vi "VM Spy - Dialog - Context Info.vi"(11 "VC Handle":T1=-1) -> (0 "update":bool)   [LabVIEW 2021]
doc: "::: CalcExpress Toolkit :::\nCopyright (c) 2000-2026 Konstantin Shifershteyn. All rights reserved."
uses:
  vi.lib/addons/CalcExpress/cetypes.llb/VarMan Context Life Time.ctl
  vi.lib/addons/CalcExpress/cetypes.llb/VarMan Variable Context Handle.ctl
panel:
  in  "calc size":bool
  in  "size utits":enum16{"Bytes", "KB", "MB"}(ring)
  out "Intended lifetime":T2
  out "used memory":dbl format="%#.3f"
  in  "destroy":bool
  in  "open VI":bool
  out "VI state":string
  out "Creator":string
  in  "close":bool
  in  "rename":bool
  out "Context name":string
  out "Context handle":i32=-1
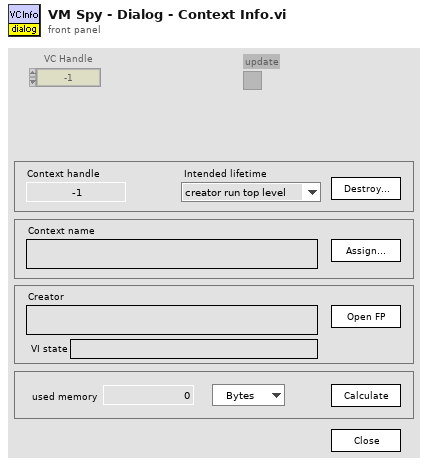
[diagram p1: front panel]
types:
  T1 = typedef "VarMan Variable Context Handle.ctl" = i32
  T2 = typedef "VarMan Context Life Time.ctl" = enum32{"creator run top level", "creator running ", "creator in memory", "untill closed"}
  T3 = enum32{"Bad", "Idle", "Run top level", "Running"}
  T4 = typedef "eventvkey.ctl" = enum16{"ASCII", "Enter", "Return", "Shift", "Ctrl", "Alt", "Cmd", "Opt", "Caps", "NumLock", "Clear", "Break", "Up", "Down", "Left", "Right", "Insert", "Delete", "Home", "End", "PageUp", "PageDown", "Escape", "Help", "Pause", "ScrollLock", "F1", "F2", "F3", "F4", "F5", "F6", "F7", "F8", "F9", "F10", "F11", "F12", "F13", "F14", "F15", "F16", "F17", "F18", "F19", "F20", "F21", "F22", "F23", "F24", "Play", "VolumeUp", "VolumeDown", "Mute", "Two Byte Char"}
  T5 = cluster{"Shift":bool, "Ctrl":bool, "Alt":bool, "Cmd":bool, "Opt":bool}
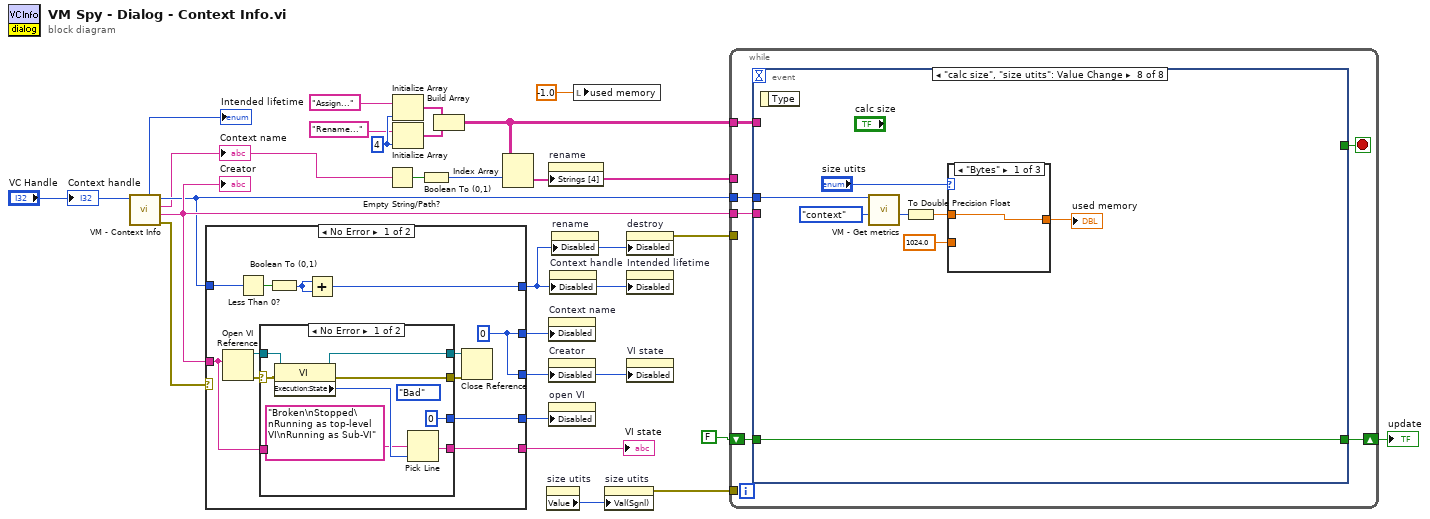
[diagram p0: block diagram]
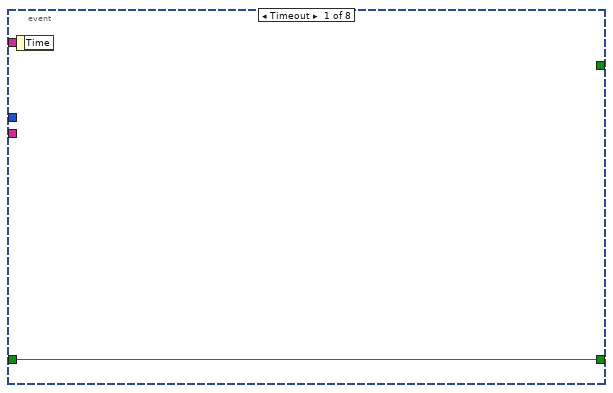
[diagram p2: hidden frame]
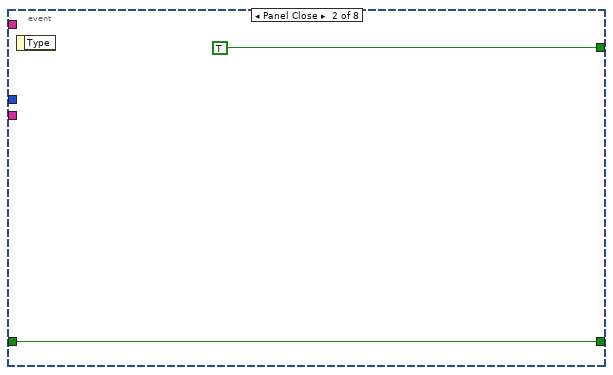
[diagram p3: hidden frame]
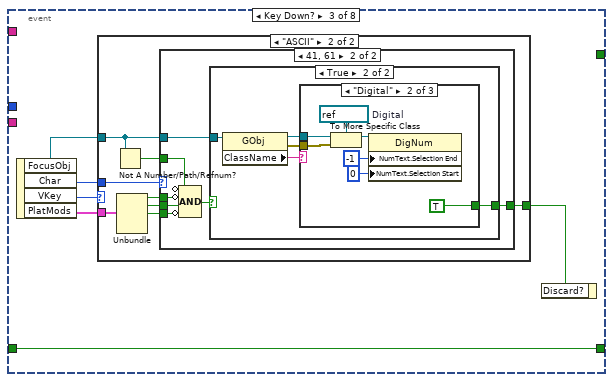
[diagram p4: hidden frame]
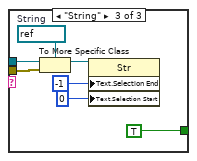
[diagram p9: hidden frame]
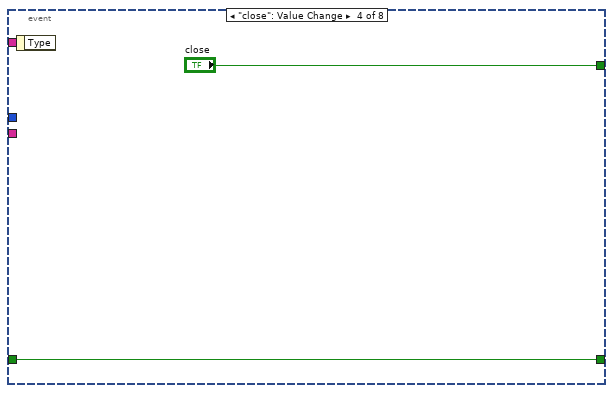
[diagram p10: hidden frame]
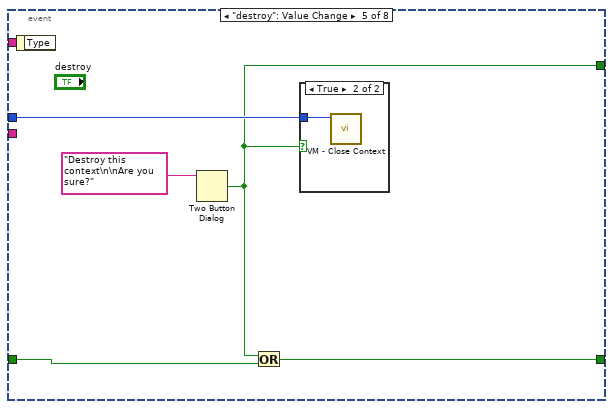
[diagram p11: hidden frame]
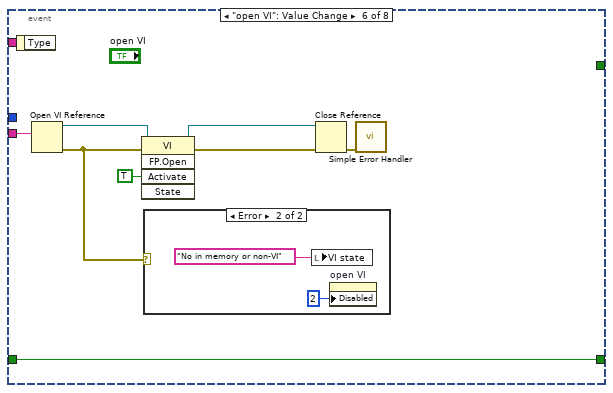
[diagram p13: hidden frame]
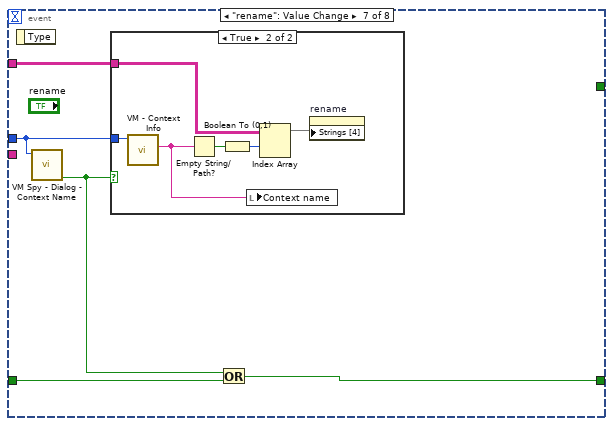
[diagram p15: hidden frame]
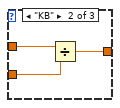
[diagram p17: hidden frame]
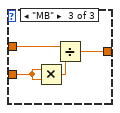
[diagram p18: hidden frame]
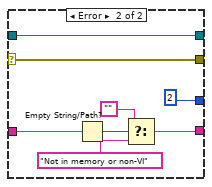
[diagram p19: hidden frame]
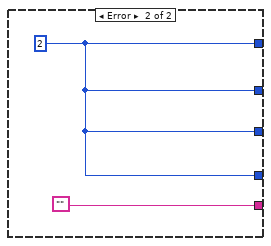
[diagram p20: hidden frame]
diagram:
  w15 = 4 ("dimension size")
  n1 = call "VM - Context Info.vi"("VC Handle"="VC Handle") -> ("error out"=w26:errorcluster, "Creator"=w20:string, "VC Name"=w16:string, "dup VC Handle"=w19:T1, "context life time"=→"Intended lifetime":T2)  [unwired: 6 in]
  "Context name" <- w16
  "Creator" <- w20
  n2 = case shown="No Error" w26 {
    tunnel: w19 -> [w35 _]
    tunnel: w20 -> [w28 _]
    tunnel: [w36 w55] -> w17
    tunnel: [w27 w55] -> w21
    tunnel: [w32 w55] -> w25
    tunnel: [w31 ""] -> w24
    tunnel: [w27 w55] -> w18
    frame No Error {
      w27 = i16 0
      n3 = Open VI Reference(vi path=w28) -> (vi reference=w34:refnum<vi>, error out=w33:errorcluster)  [unwired: 5 in]
      n4 = Less Than 0?(x=w35) -> (x < 0?=w38:bool)
      n5 = case shown="No Error" w33 {
        selector: w33 -> [w45 w52]
        tunnel: w34 -> [w46 w53]
        tunnel: [i16 0 i16 2] -> w32
        tunnel: [w41 w51] -> w31
        tunnel: [w40 w53] -> w30
        tunnel: [w39 w52] -> w29
        tunnel: w28 -> [_ w48]
        frame No Error {
          (unwired) T3."Bad" ("Execution:State")
          n6 = property class="VI"(reference=w46, error in=w45) -> (reference out=w40:refnum<vi>, error out=w39:errorcluster, "Execution:State"=w43:T3)
          n7 = Pick Line(multi-line string="Broken\nStopped\nRunning as top-level VI\nRunning as Sub-VI", line index=w43) -> (output string=w41:string)  [unwired: 1 in]
        }
        frame Error {
          n8 = Empty String/Path?(string/path=w48) -> (empty?=w50:bool)
          n9 = Select(t="", s=w50, f="Not in memory or non-VI") -> (s? t:f=w51:string)
        }
      }
      n10 = Boolean To (0,1)(Boolean=w38) -> (0, 1=w37:i16)
      n11 = Add(x=w37, y=w37) -> (x+y=w36:i16)
      n12 = Close Reference(reference=w30, error in (no error)=w29) -> ()  [unwired: 1 out]
    }
    frame Error {
      w55 = i16 2
    }
  }
  "VI state" <- w24
  n13 = Empty String/Path?(string/path=w16) -> (empty?=w10:bool)
  n14 = Initialize Array("Assign...", w15) -> (w12:string[])
  n15 = Initialize Array("Rename...", w15) -> (w11:string[])
  n16 = Boolean To (0,1)(Boolean=w10) -> (0, 1=w9:i16)
  n17 = Build Array(w12, w11) -> (w7:string[][])
  n18 = Index Array(array=w7, index (row)=w9) -> (element=w8:string[])  [unwired: 1 in]
  n19 = property on="size utits" class="Enum (strict)"() -> ("Value"=w3:enum16{"Bytes", "KB", "MB"})  [unwired: 2 in, 2 out]
  n20 = property on="rename" class="Bool"("Strings [4]"=w8) -> ()  [unwired: 2 in, 2 out]
  n21 = property on="Context name" class="Str"("Disabled"=w18) -> ()  [unwired: 2 in, 2 out]
  n22 = property on="Creator" class="Str"("Disabled"=w21) -> ()  [unwired: 2 in, 2 out]
  n23 = property on="open VI" class="Bool"("Disabled"=w25) -> ()  [unwired: 2 in, 2 out]
  n24 = property on="Context handle" class="DigNum (strict)"("Disabled"=w17) -> ()  [unwired: 2 in, 2 out]
  n25 = property on="rename" class="Bool"("Disabled"=w17) -> ()  [unwired: 2 in, 2 out]
  n26 = local write "used memory"(-1.0 ("used memory")) -> ()
  n27 = property on="size utits" class="Enum (strict)"("Val(Sgnl)"=w3) -> (error out=w2:errorcluster)  [unwired: 2 in, 1 out]
  n28 = property on="destroy" class="Bool"("Disabled"=w17) -> (error out=w1:errorcluster)  [unwired: 2 in, 1 out]
  n29 = property on="Intended lifetime" class="Enum (strict)"("Disabled"=w17) -> ()  [unwired: 2 in, 2 out]
  n30 = property on="VI state" class="Str"("Disabled"=w21) -> ()  [unwired: 2 in, 2 out]
  n31 = while {
    shift-right: [w60] -> w22
    shift-left: FALSE -> [w61]
    tunnel: w20 -> [w58]
    tunnel: w19 -> [w59]
    tunnel: w8 -> [_]
    tunnel: w7 -> [w57]
    tunnel: w2 -> [_]
    tunnel: w1 -> [_]
    stop <- w62 stop-if-true
    n32 = event shown="[7] \"calc size\", \"size utits\": Value Change" {
      selector: _ -> [_ _ _ _ _ _ _ _]
      dyn-events: _ -> [_ _ _ _ _ _ _ _]
      timeout: _ -> [_ _ _ _ _ _ _ _]
      tunnel: [_ TRUE _ "close" w109 _ _ _] -> w62
      tunnel: w61 -> [w63 w64 w71 w106 w108 w121 w127 w140]
      tunnel: [w63 w64 w71 w106 w110 w121 w128 w140] -> w60
      tunnel: w59 -> [_ _ _ _ w111 _ w125 w142]
      tunnel: w58 -> [_ _ _ _ _ w120 _ _]
      tunnel: w57 -> [_ _ _ _ _ _ w124 _]
      event Timeout {
        n33 = event-data() -> ()  [unwired: 1 in, 1 out]
      }
      event Panel Close {
        n34 = event-data() -> ()  [unwired: 1 in, 1 out]
      }
      event Key Down? {
        n35 = event-data() -> ("FocusObj"=w67:refnum<vi>, "Char"=w68:i16, "VKey"=w69:T4, "PlatMods"=w70:T5)  [unwired: 1 in]
        n36 = case shown="\"ASCII\"" w69 {
          tunnel: w70 -> [_ w79]
          tunnel: [_ w73] -> w66
          tunnel: w68 -> [_ w75]
          tunnel: w67 -> [_ w74]
          frame Default {
          }
          frame "ASCII" {
            n37 = Not A Number/Path/Refnum?(number/path/refnum=w74) -> (NaN/Path/Refnum?=w72:bool)
            n38 = Unbundle(w79) -> ("Shift"=w78:bool, "Ctrl"=w77:bool, "Alt"=w76:bool)  [unwired: 2 out]
            n39 = case shown="41, 61" w75 {
              tunnel: w78 -> [_ w86]
              tunnel: w77 -> [_ w85]
              tunnel: w76 -> [_ w84]
              tunnel: w74 -> [_ w82]
              tunnel: [_ w81] -> w73
              tunnel: w72 -> [_ w80]
              frame Default {
              }
              frame 65, 97 {
                n40 = Compound Arithmetic op=AND(invert w80, invert w86, w85, invert w84) -> (w83:bool)
                n41 = case shown="True" w83 {
                  tunnel: w82 -> [_ w91]
                  tunnel: [_ w89] -> w81
                  frame False {
                  }
                  frame True {
                    n42 = property class="GObj"(reference=w91) -> (reference out=w88:refnum<vi>, error out=w87:errorcluster, "ClassName"=w90:string)  [unwired: 1 in]
                    n43 = case shown="\"Digital\"" w90 {
                      tunnel: [_ TRUE TRUE] -> w89
                      tunnel: w88 -> [_ w96 w103]
                      tunnel: w87 -> [_ w95 w102]
                      frame Default {
                      }
                      frame "Digital" {
                        w97 = refnum<vi> refnum  # Digital
                        n44 = To More Specific Class(target class=w97, reference=w96, error in=w95) -> (specific class reference=w94:refnum<vi>)  [unwired: 1 out]
                        n45 = property class="DigNum"(reference=w94, "NumText.Selection End"=-1 ("Numeric Text.Selection:End"), "NumText.Selection Start"=u32 0 ("Numeric Text.Selection:Start")) -> ()  [unwired: 1 in, 2 out]
                      }
                      frame "String" {
                        w104 = refnum<vi> refnum  # String
                        n46 = To More Specific Class(target class=w104, reference=w103, error in=w102) -> (specific class reference=w101:refnum<vi>)  [unwired: 1 out]
                        n47 = property class="Str"(reference=w101, "Text.Selection End"=-1 ("Numeric Text.Selection:End"), "Text.Selection Start"=u32 0 ("Numeric Text.Selection:Start")) -> ()  [unwired: 1 in, 2 out]
                      }
                    }
                  }
                }
              }
            }
          }
        }
        n48 = event-data("Discard?"=w66) -> ()  [unwired: 1 in, 1 out]
      }
      event "close": Value Change {
        n49 = event-data() -> ()  [unwired: 1 in, 1 out]
      }
      event "destroy": Value Change {
        n50 = event-data() -> ()  [unwired: 1 in, 1 out]
        n51 = Two Button Dialog(message="Destroy this context\n\nAre you sure?") -> (T button?=w109:bool)  [unwired: 2 in]
        n52 = Or(x=w109, y=w108) -> (x .or. y?=w110:bool)
        n53 = case shown="True" w109 {
          tunnel: w111 -> [_ w113]
          frame False {
          }
          frame True {
            n54 = call "VM - Close Context.vi"("VC Handle"=w113) -> ()  [unwired: 9 in, 2 out]
          }
        }
      }
      event "open VI": Value Change {
        n55 = event-data() -> ()  [unwired: 1 in, 1 out]
        n56 = Open VI Reference(vi path=w120) -> (vi reference=w119:refnum<vi>, error out=w115:errorcluster)  [unwired: 5 in]
        n57 = invoke class="VI" method="FP.Open"(reference=w119, error in=w115, "Activate"=TRUE ("Activate?")) -> (reference out=w118:refnum<vi>, error out=w117:errorcluster)  [unwired: 2 in, 3 out]
        n58 = case shown="Error" w115 {
          frame No Error {
          }
          frame Error {
            n59 = local write "VI state"("No in memory or non-VI") -> ()
            n60 = property on="open VI" class="Bool"("Disabled"=u8 2) -> ()  [unwired: 2 in, 2 out]
          }
        }
        n61 = Close Reference(reference=w118, error in (no error)=w117) -> (error out=w116:errorcluster)
        n62 = call <vilib>:"Simple Error Handler.vi"("error in (no error)"=w116) -> ()  [unwired: 4 in, 5 out]
      }
      event "rename": Value Change {
        n63 = event-data() -> ()  [unwired: 1 in, 1 out]
        n64 = call "VM Spy - Dialog - Context Name.vi"("VC Handle"=w125) -> ("OK out"=w126:bool)  [unwired: 9 in, 1 out]
        n65 = case shown="True" w126 {
          tunnel: w125 -> [_ w134]
          tunnel: w124 -> [_ w129]
          frame False {
          }
          frame True {
            n66 = call "VM - Context Info.vi"("VC Handle"=w134) -> ("VC Name"=w132:string)  [unwired: 6 in, 4 out]
            n67 = Empty String/Path?(string/path=w132) -> (empty?=w131:bool)
            n68 = Boolean To (0,1)(Boolean=w131) -> (0, 1=w130:i16)
            n69 = local write "Context name"(w132) -> ()
            n70 = Index Array(array=w129, index (row)=w130) -> (element=w133:string[])  [unwired: 1 in]
            n71 = property on="rename" class="Bool"("Strings [4]"=w133) -> ()  [unwired: 2 in, 2 out]
          }
        }
        n72 = Or(x=w126, y=w127) -> (x .or. y?=w128:bool)
      }
      event "calc size", "size utits": Value Change {
        n73 = event-data() -> ()  [unwired: 1 in, 1 out]
        n74 = call "VM - Get metrics.vi"("object"=enum32{"variable", "context", "total"}."context", "VC Handle"=w142) -> ("total size, bytes"=w138:u64)  [unwired: 5 in, 4 out]
        n75 = To Double Precision Float(number=w138) -> (double precision float=w135:dbl)
        n76 = case shown="\"Bytes\"" "size utits" {
          tunnel: w135 -> [w143 w146 w150]
          tunnel: 1024.0 ("y") -> [_ w145 w149]
          tunnel: [w143 w144 w147] -> w136
          frame "Bytes" {
          }
          frame "KB" {
            n77 = Divide(x=w146, y=w145) -> (x/y=w144:dbl)
          }
          frame "MB" {
            n78 = Multiply(x=w149, y=w149) -> (x*y=w148:dbl)
            n79 = Divide(x=w150, y=w148) -> (x/y=w147:dbl)
          }
        }
        "used memory" <- w136
      }
    }
  }
  "update" <- w22
  "Context handle" <- "VC Handle"
